vi "Move Turn Table.vi"(8 "error in (no error)":errorcluster, 11 "AUDIX EM1000 in":refnum<class "AUDIX EM1000.lvclass">) -> (0 "error out":errorcluster, 3 "AUDIX EM1000 out":refnum<class "AUDIX EM1000.lvclass">)   [LabVIEW 2023, in "Turn Table and Mast.lvlib" / "AUDIX EM1000.lvclass"]
uses:
  AUDIX EM1000.lvclass
  AUDIX EM1000.lvclass/AUDIX EM1000.ctl
panel:
  out "VISA resource name out":refnum<visa-resource-name>
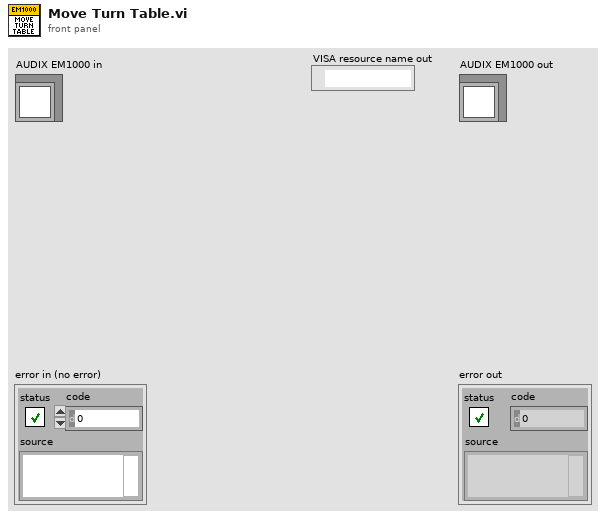
[diagram p1: front panel]
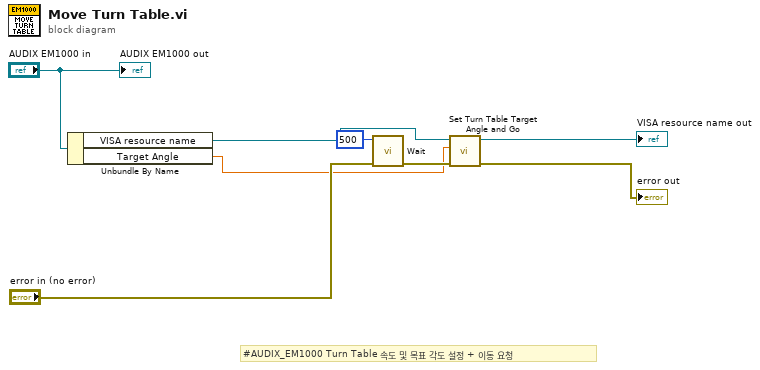
[diagram p0: block diagram]
diagram:
  # "#AUDIX_EM1000 Turn Table 속도 및 목표 각도 설정 + 이동 요청"
  n1 = Unbundle By Name("AUDIX EM1000 in") -> ("VISA resource name"=w3:refnum<visa-resource-name>, "Target Angle"=w2:dbl)
  n2 = call "Wait.vi"("에러 상수 입력"="error in (no error)", "대기 시간 (ms)"=u32 500) -> ("에러 상수 출력"=w6:errorcluster)  [unwired: 9 in]
  n3 = call "Set Turn Table Target Angle and Go.vi"("error in (no error)"=w6, "Target Angle"=w2, "VISA Refnum in"=w3) -> ("error out"=→"error out":errorcluster, "VISA Refnum out"=→"VISA resource name out":refnum<visa-resource-name>)  [unwired: 7 in]
  "AUDIX EM1000 out" <- "AUDIX EM1000 in"
